vi "SOS_State_Adapter.vi"(0 "error in (no error)":errorcluster caption="错误输入（无错误）", 2 "Current State":T1, 3 "Reset Timer":bool, 4 "SOS Pressed":bool) -> (1 "error out":errorcluster caption="错误输出", 5 "State To Machine":T1, 6 "SOS Held Milliseconds":u32, 7 "SOS Requested":bool)   [LabVIEW 2020]
doc: "PLACEHOLDER: error interface only. Alarm simulation NOT implemented."
uses:
  Controls/State.ctl
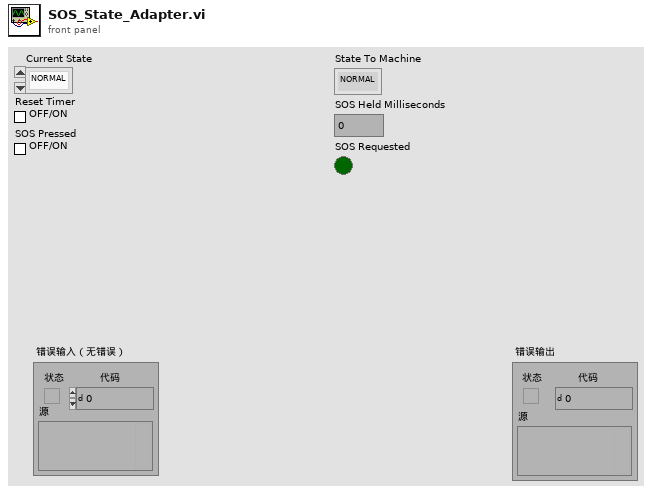
[diagram p1: front panel]
types:
  T1 = typedef "State.ctl" = enum16{"NORMAL", "SUSPECT", "COUNTDOWN", "ALARM", "RESET"}
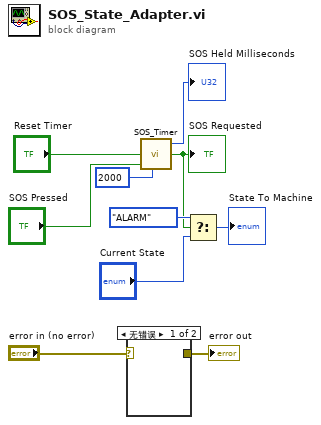
[diagram p0: block diagram]
diagram:
  n1 = case shown="无错误" "error in (no error)" {
    selector: "error in (no error)" -> [_ w11]
    tunnel: [_ w11] -> w9
    frame No Error {
    }
    frame Error {
    }
  }
  "error out" <- w9
  n2 = call "SOS_Timer.vi"("Reset Timer"="Reset Timer", "Pressed"="SOS Pressed", "Required Milliseconds"=u32 2000) -> ("Held Milliseconds"=→"SOS Held Milliseconds":u32, "SOS Requested"=w3:bool)  [unwired: 2 in, 1 out]
  "SOS Requested" <- w3
  n3 = Select(t=State."ALARM", s=w3, f="Current State") -> (s? t:f=→"State To Machine":T1)
